vi "TCP Server Destroy.vi"(8 "error in (no error)":errorcluster, 11 "TCP Server":refnum<class "JKI TCP Server.lvclass">) -> (0 "error out":errorcluster)   [LabVIEW 2020, in "JKI TCP Server.lvclass"]
uses:
  JKI TCP Server.lvclass
  JKI TCP Server.lvclass/JKI TCP Server.ctl
panel:
  # "Copyright © 2004-2008 JKI. All rights reserved.\n\nAuthor: Jim Kring [jim.kring@jameskring.com]\n\nThis library is provided \"AS IS\" ,WITHOUT WARRANTIES OR \nCONDITIONS OF ANY KIND, either express or implied.\n\nJames Kring, Inc. -- http://www.jameskring.com"
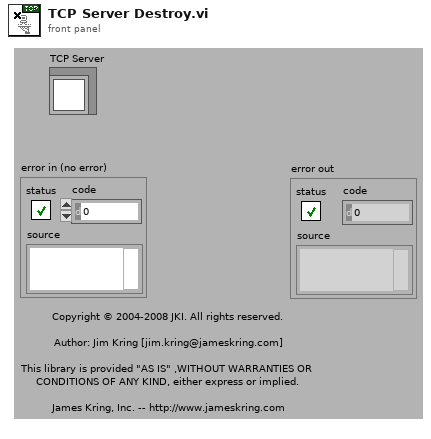
[diagram p1: front panel]
types:
  T1 = typedef "JKI TCP Server.lvclass/TCP Server Data.ctl" = cluster{"Listener Info":T2, "Connection Process VI RefNums":refnum<vi>[], "dup connection IDs (for quick search)":refnum<k5>[], "Connections":T3[], "Connection Handler VI Path":path, "Handler Is Reentrant?":bool, "TCP Handler Instance RefNums":T4[], "TCP Handler VI RefNum":T4, "No. Connections":u32, "Max Connections":u32, "server start time":u32, "Additional Data":variant}
  T2 = typedef "JKI TCP Server.lvclass/TCP Server Listener Info Cluster.ctl" = cluster{"listener ID":refnum<k5>, "net address":u32, "port":u16, "Listener Process VI Refnum":refnum<vi>}
  T3 = typedef "JKI TCP Server.lvclass/TCP Server Connection Info Cluster.ctl" = cluster{"connection ID":refnum<k5>, "Remote Address":string, "remote port":u16, "connection start time":u32}
  T4 = typedef "JKI TCP Server.lvclass/TCP Server Handler RefNum.ctl" = refnum<vi>
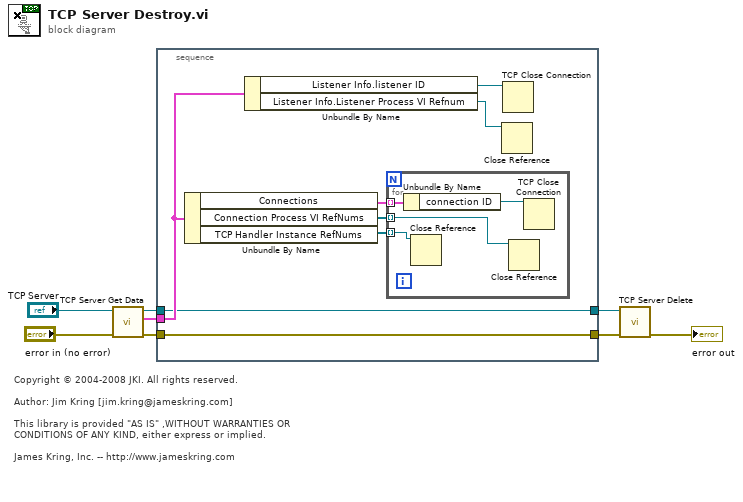
[diagram p0: block diagram]
diagram:
  # "Copyright © 2004-2008 JKI. All rights reserved.\n\nAuthor: Jim Kring [jim.kring@jameskring.com]\n\nThis library is provided \"AS IS\" ,WITHOUT WARRANTIES OR \nCONDITIONS OF ANY KIND, either express or implied.\n\nJames Kring, Inc. -- http://www.jameskring.com"
  n1 = call "TCP Server Get Data.vi"("error in (no error)"="error in (no error)", "RefNum"="TCP Server") -> ("error out"=w3:errorcluster, "Data out"=w5:T1, "dup RefNum"=w4:refnum<class "JKI TCP Server.lvclass">)  [unwired: 7 in]
  n2 = stacked-sequence {
    tunnel: w5 -> [w15]
    tunnel: w4 -> [w10]
    tunnel: w3 -> [w11]
    tunnel: [w11] -> w2
    tunnel: [w10] -> w1
    frame #0 {
      n3 = Unbundle By Name(w15) -> ("Connections"=w14:T3[], "Connection Process VI RefNums"=w13:refnum<vi>[], "TCP Handler Instance RefNums"=w9:T4[])
      n4 = Unbundle By Name(w15) -> ("Listener Info.listener ID"=w16:refnum<k5>, "Listener Info.Listener Process VI Refnum"=w12:refnum<vi>)
      n5 = for {
        tunnel: w14 -> [w20] mode=indexing
        tunnel: w13 -> [w18] mode=indexing
        tunnel: w9 -> [w17] mode=indexing
        n6 = Unbundle By Name(w20) -> ("connection ID"=w19:refnum<k5>)
        n7 = Close Reference(reference=w17) -> ()  [unwired: 1 in, 1 out]
        n8 = Close Reference(reference=w18) -> ()  [unwired: 1 in, 1 out]
        n9 = TCP Close Connection(connection ID=w19) -> ()  [unwired: 2 in, 2 out]
      }
      n10 = Close Reference(reference=w12) -> ()  [unwired: 1 in, 1 out]
      n11 = TCP Close Connection(connection ID=w16) -> ()  [unwired: 2 in, 2 out]
    }
  }
  n12 = call "TCP Server Delete.vi"("error in (no error)"=w2, "TCP Server"=w1) -> ("error out"=→"error out":errorcluster)  [unwired: 9 in]
